vi "SeqEditor_StepMLSTDrop.vi"(7 "内部拖拽":bool, 9 "Ctrl":bool, 10 "Coords":T1, 11 "CtlRef":refnum<vi>) -> (0 "error out":errorcluster, 3 "CtlRef 2":refnum<vi>)   [LabVIEW 2017, in "NLTest.lvclass"]
uses:
  NLTest.lvclass
  <vilib>/Utility/miscctls.llb/LVPoint32TypeDef.ctl
panel:
  # "BY Ytester"
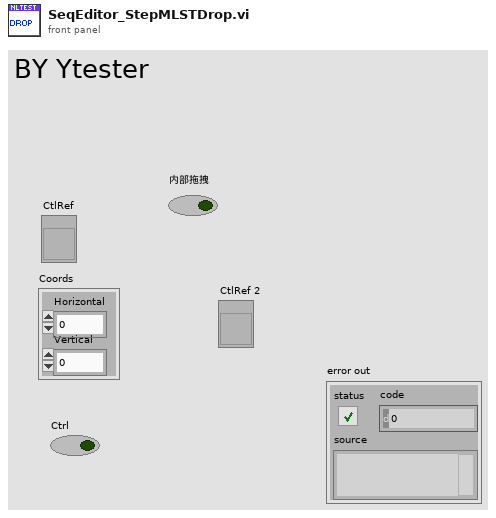
[diagram p1: front panel]
types:
  T1 = typedef "LVPoint32TypeDef.ctl" = cluster{"Horizontal":i32, "Vertical":i32}
  T2 = typedef "LVRowAndColumnTypeDef.ctl" = cluster{"Row":i32, "Column":i32}
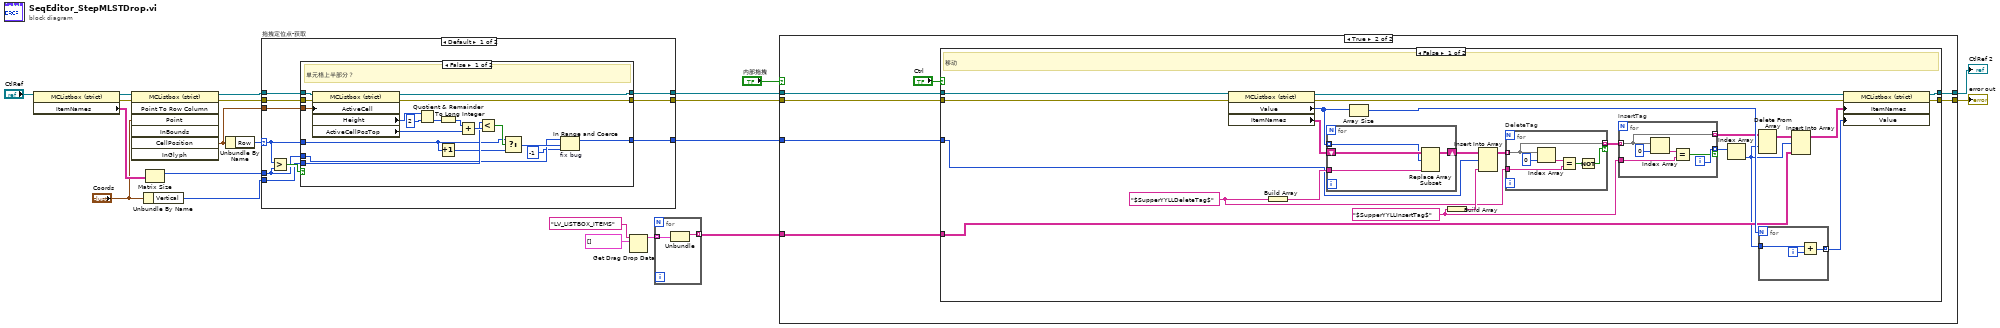
[diagram p0: block diagram]
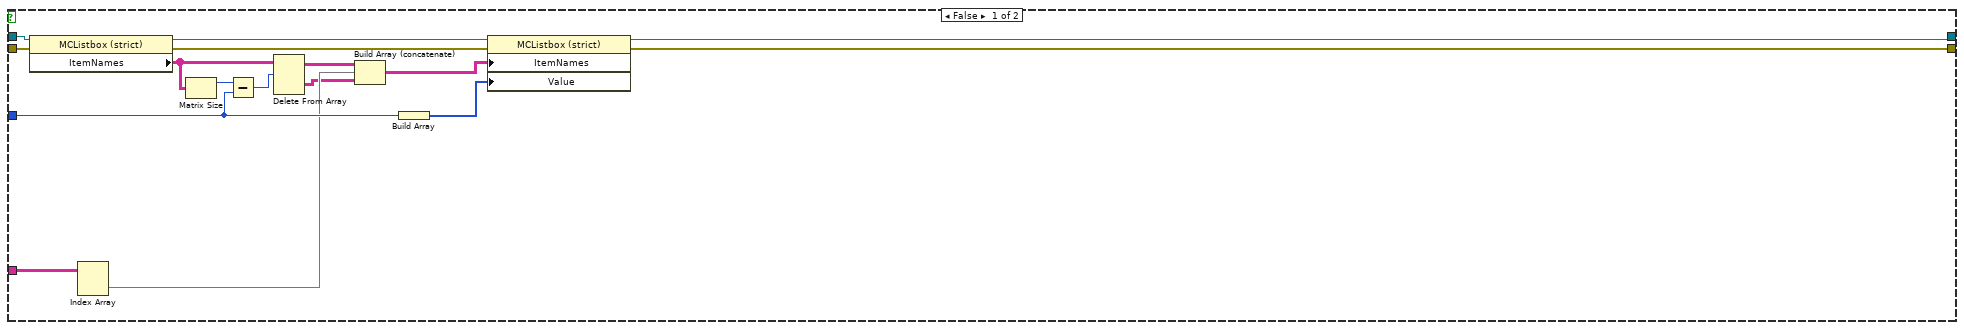
[diagram p2: hidden frame]
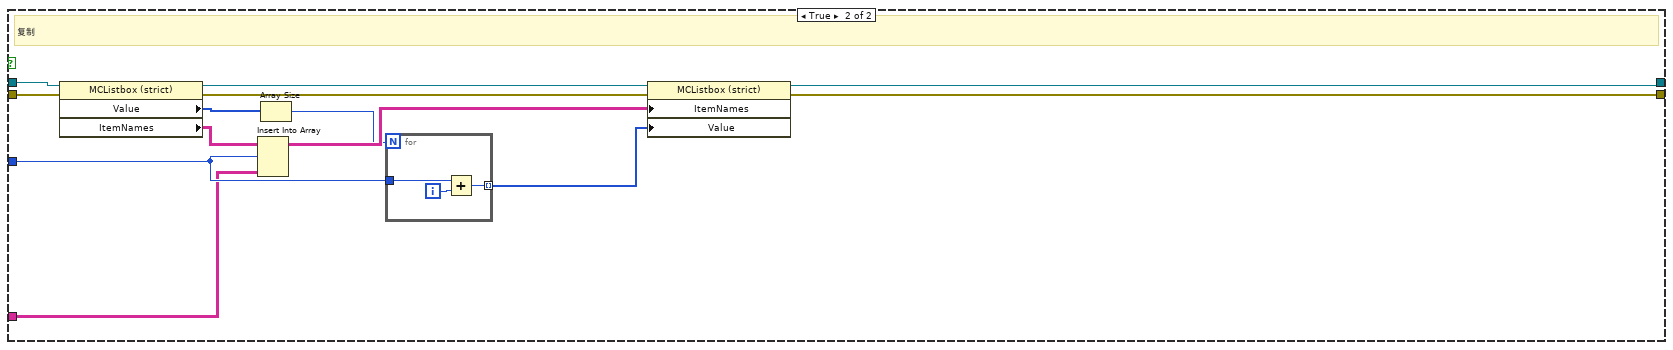
[diagram p3: hidden frame]
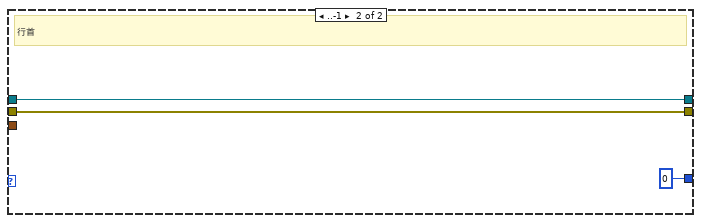
[diagram p5: hidden frame]
diagram:
  n1 = property class="MCListbox (strict)"(reference="CtlRef") -> (reference out=w12:refnum<vi>, error out=w7:errorcluster, "ItemNames"=w14:string[][])  [unwired: 1 in]
  n2 = invoke class="MCListbox (strict)" method="Point To Row Column"(reference=w12, error in=w7, "Point"="Coords") -> (reference out=w19:refnum<vi>, error out=w6:errorcluster, "CellPosition"=w18:T2)  [unwired: 4 in, 4 out]
  n3 = Unbundle By Name("Coords") -> ("Vertical"=w17:i32)
  n4 = Matrix Size(0:w14) -> (1:w16:i32)  [unwired: 1 out]
  n5 = Unbundle By Name(w18) -> ("Row"=w15:i32)
  n6 = case "拖拽定位点-获取" shown="Default" w15 {
    selector: w15 -> [w28 _]
    tunnel: [w30 0] -> w21
    tunnel: w16 -> [w29 _]
    tunnel: w17 -> [w27 _]
    tunnel: w18 -> [w26 _]
    tunnel: w19 -> [w25 w55]
    tunnel: [w24 w55] -> w20
    tunnel: w6 -> [w23 w54]
    tunnel: [w22 w54] -> w5
    frame Default {
      n7 = Greater?(x=w28, y=w29) -> (0:w31:bool)
      n8 = case shown="False" w31 {
        tunnel: [w34 w53] -> w30
        tunnel: w29 -> [w33 w53]
        tunnel: w28 -> [w39 _]
        tunnel: w27 -> [w44 _]
        tunnel: w26 -> [w43 _]
        tunnel: w25 -> [w42 w52]
        tunnel: [w41 w52] -> w24
        tunnel: w23 -> [w37 w51]
        tunnel: [w36 w51] -> w22
        frame False {
          # "单元格上半部分？"
          n9 = property class="MCListbox (strict)"(reference=w42, error in=w37, "ActiveCell"=w43) -> (reference out=w41:refnum<vi>, error out=w36:errorcluster, "Height"=w45:u32, "ActiveCellPosTop"=w48:i32)
          n10 = Quotient & Remainder(x=w45, y=u32 2) -> (floor(x/y)=w47:u32)  [unwired: 1 out]
          n11 = To Long Integer(number=w47) -> (32bit integer=w49:i32)
          n12 = Increment(x=w39) -> (x+1=w38:i32)
          n13 = Add(x=w49, y=w48) -> (x+y=w50:i32)
          n14 = Less?(x=w44, y=w50) -> (x < y?=w40:bool)
          n15 = Select(t=w39, s=w40, f=w38) -> (s? t:f=w35:i32)
          n16 = In Range and Coerce "fix bug"(upper limit=w33, x=w35, lower limit=-1) -> (coerced(x)=w34:i32)  [unwired: 1 out]
        }
        frame True {
          # "最大空白处"
        }
      }
    }
    frame ..-1 {
      # "行首"
    }
  }
  n17 = Get Drag Drop Data(8:cluster{string[], i32}[] [] ("appended array"), 9:"LV_LISTBOX_ITEMS" ("data name")) -> (3:w10:cluster{string[], i32}[])  [unwired: 1 in, 1 out]
  n18 = for {
    tunnel: w10 -> [w58] mode=indexing
    tunnel: [w57] -> w3 mode=indexing
    n19 = Unbundle(w58) -> (w57:string[])  [unwired: 1 out]
  }
  n20 = case shown="True" "内部拖拽" {
    tunnel: w21 -> [w65 w81]
    tunnel: w20 -> [w69 w80]
    tunnel: w5 -> [w68 w79]
    tunnel: [w67 w78] -> w4
    tunnel: w3 -> [w70 w77]
    tunnel: [w66 w75] -> w2
    frame False {
      n21 = property class="MCListbox (strict)"(reference=w69, error in=w68) -> (reference out=w74:refnum<vi>, error out=w71:errorcluster, "ItemNames"=w73:string[][])
      n22 = Index Array(array=w70) -> (element=w63:string[])  [unwired: 2 in]
      n23 = Matrix Size(0:w73) -> (1:w62:i32)  [unwired: 1 out]
      n24 = Subtract(x=w62, y=w65) -> (x-y=w61:i32)
      n25 = Delete From Array(array=w73, length=w61) -> (deleted portion=w59:string[][], array with subset deleted=w60:string[][])  [unwired: 2 in]
      n26 = Build Array (concatenate)(w60, w63, w59) -> (w64:string[][])
      n27 = Build Array(w65) -> (w72:i32[])
      n28 = property class="MCListbox (strict)"(reference=w74, error in=w71, "ItemNames"=w64, "Value"=w72) -> (reference out=w67:refnum<vi>, error out=w66:errorcluster)
    }
    frame True {
      n29 = case shown="False" "Ctrl" {
        tunnel: w80 -> [w105 w136]
        tunnel: w77 -> [w90 w125]
        tunnel: w81 -> [w97 w131]
        tunnel: w79 -> [w85 w129]
        tunnel: [w83 w127] -> w75
        tunnel: [w82 w126] -> w78
        frame False {
          w93 = "$SupperYYLLInsertTag$"
          w95 = "$SupperYYLLDeleteTag$"
          # "移动"
          n30 = property class="MCListbox (strict)"(reference=w105, error in=w85) -> (reference out=w102:refnum<vi>, error out=w84:errorcluster, "Value"=w100:i32[], "ItemNames"=w104:string[][])
          n31 = Build Array(w95) -> (w103:string[])
          n32 = for {
            shift-right: [w123] -> w96
            shift-left: w104 -> [w124]
            tunnel: w100 -> [w122] mode=indexing
            tunnel: w103 -> [w121]
            n33 = Replace Array Subset(array=w124, new element=w121, index (row)=w122) -> (w123:string[][])  [unwired: 1 in]
          }
          n34 = Array Size(array=w100) -> (size(s)=w101:i32)
          n35 = Build Array(w93) -> (w98:string[])
          n36 = Insert Into Array(array=w96, index (row)=w97, new element=w98) -> (w86:string[][])  [unwired: 1 in]
          n37 = for "DeleteTag" {
            tunnel: w86 -> [w115] mode=indexing
            tunnel: w95 -> [w116]
            tunnel: [w115] -> w94 mode=indexing if=w113
            n38 = Index Array(array=w115, index=0) -> (element=w112:string)
            n39 = Equal?(x=w112, y=w116) -> (x = y?=w114:bool)
            n40 = Not(x=w114) -> (.not. x?=w113:bool)
          }
          n41 = for "InsertTag" {
            tunnel: w94 -> [w108] mode=indexing
            tunnel: w93 -> [w110]
            tunnel: [w108] -> w91 mode=indexing
            tunnel: [w107] -> w88 mode=indexing if=w106
            i -> [w107]
            n42 = Index Array(array=w108, index=0) -> (element=w109:string)
            n43 = Equal?(x=w109, y=w110) -> (x = y?=w106:bool)
          }
          n44 = Index Array(array=w88) -> (element=w87:i32)  [unwired: 1 in]
          n45 = Delete From Array(array=w91, index (row)=w87) -> (array with subset deleted=w92:string[][])  [unwired: 2 in, 1 out]
          n46 = for {
            N: w101 -> [_]
            tunnel: [w119] -> w99 mode=indexing
            tunnel: w87 -> [w118]
            i -> [w120]
            n47 = Add(x=w118, y=w120) -> (x+y=w119:i32)
          }
          n48 = Insert Into Array(array=w92, index (row)=w87, new element=w90) -> (w89:string[][])  [unwired: 1 in]
          n49 = property class="MCListbox (strict)"(reference=w102, error in=w84, "ItemNames"=w89, "Value"=w99) -> (reference out=w82:refnum<vi>, error out=w83:errorcluster)
        }
        frame True {
          # "复制"
          n50 = property class="MCListbox (strict)"(reference=w136, error in=w129) -> (reference out=w137:refnum<vi>, error out=w128:errorcluster, "Value"=w133:i32[], "ItemNames"=w135:string[][])
          n51 = Insert Into Array(array=w135, index (row)=w131, new element=w125) -> (w134:string[][])  [unwired: 1 in]
          n52 = Array Size(array=w133) -> (size(s)=w132:i32)
          n53 = for {
            N: w132 -> [_]
            tunnel: w131 -> [w139]
            tunnel: [w138] -> w130 mode=indexing
            i -> [w140]
            n54 = Add(x=w139, y=w140) -> (x+y=w138:i32)
          }
          n55 = property class="MCListbox (strict)"(reference=w137, error in=w128, "ItemNames"=w134, "Value"=w130) -> (reference out=w126:refnum<vi>, error out=w127:errorcluster)
        }
      }
    }
  }
  "CtlRef 2" <- w4
  "error out" <- w2
